vi "Comparaison alarmes 1 2 3 4.vi"() -> (2 "AL OK nouveau":cluster{"AL OK 1 COM":u16[]}[](array[cluster]) {"AL OK 1 COM" items=["data = AL", "data pas nombre", "data diff. AL"]}, 3 "problème":string, 4 "regs pb":string[](array[string]), 5 "Dépassement seuil":T1(array[cluster]))   [LabVIEW 2022 SP3]
uses:
  Variables globales/Variables glob EUROTHERM.vi
panel:
  # "COMPARAISON"
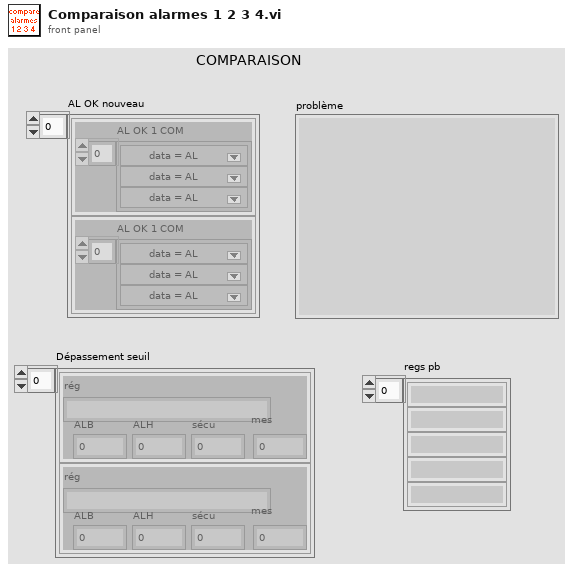
[diagram p1: front panel]
types:
  T1 = cluster{"rég":string, "mes":dbl, "ALB":dbl, "ALH":dbl, "sécu":dbl}[]
  T2 = cluster{"Noms voies select acqui 1COM":string[]}[]
  T3 = cluster{"rég":string, "mes":dbl, "ALB":dbl, "ALH":dbl, "sécu":dbl}
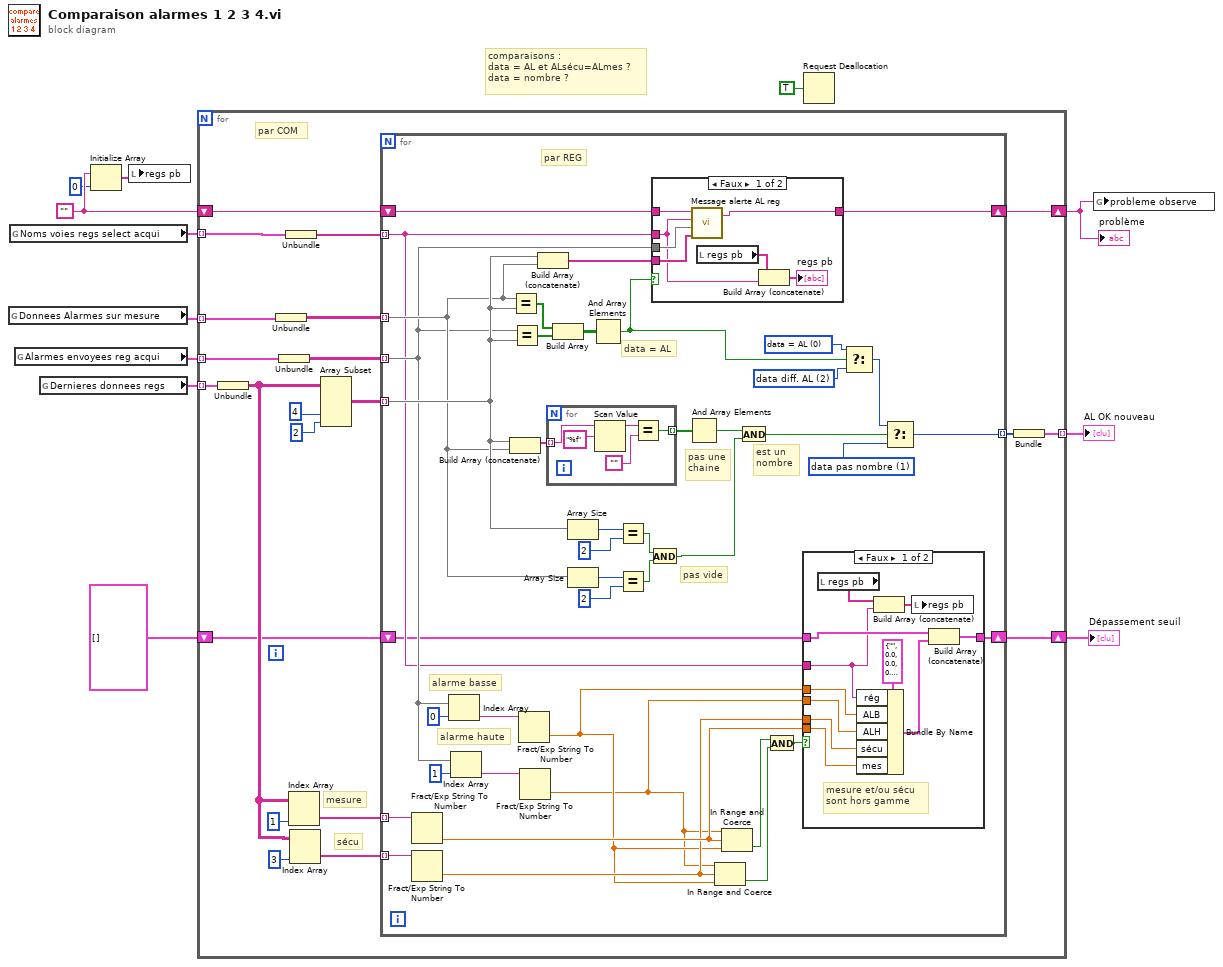
[diagram p0: block diagram]
diagram:
  w3 = ""
  # "comparaisons :\ndata = AL et ALsécu=ALmes ?\ndata = nombre ?"
  n1 = global read "Variables glob EUROTHERM.vi" "Donnees Alarmes sur mesure"() -> (w6:cluster{"AL sur mes 1COM":string[][]}[])
  n2 = global read "Variables glob EUROTHERM.vi" "Noms voies regs select acqui"() -> (w9:T2)
  n3 = global read "Variables glob EUROTHERM.vi" "Alarmes envoyees reg acqui"() -> (w11:cluster{"alarmes 1COM reg":string[][]}[])
  n4 = global read "Variables glob EUROTHERM.vi" "Dernieres donnees regs"() -> (w12:cluster{"Dernieres donnees 1COM":string[][]}[])
  n5 = Initialize Array(w3, 0 ("taille de la dimension")) -> (w2:string[])
  n6 = local write "regs pb"(w2) -> ()
  n7 = for {
    tunnel: w11 -> [w31] mode=indexing
    tunnel: w12 -> [w30] mode=indexing
    tunnel: w9 -> [w27] mode=indexing
    shift-right: [w24] -> w8
    shift-left: w3 -> [w25]
    tunnel: [w22] -> w7 mode=indexing
    tunnel: w6 -> [w21] mode=indexing
    shift-right: [w15] -> w5
    shift-left: T1 [] ("Dépassement seuil") -> [w16]
    # "sécu"
    # "mesure"
    # "par COM"
    n8 = Unbundle(w30) -> ("Dernieres donnees 1COM"=w19:string[][])
    n9 = Unbundle(w21) -> ("AL sur mes 1COM"=w20:string[][])
    n10 = Unbundle(w31) -> ("alarmes 1COM reg"=w29:string[][])
    n11 = Unbundle(w27) -> ("Noms voies select acqui 1COM"=w26:string[])
    n12 = Index Array(array=w19, index (col)=1 ("indice (ligne)")) -> (element=w18:string[])  [unwired: 1 in]
    n13 = Index Array(array=w19, index (col)=3 ("indice (ligne)")) -> (element=w17:string[])  [unwired: 1 in]
    n14 = Array Subset(array=w19, index (col)=4 ("indice"), length (col)=2 ("longueur")) -> (w28:string[][])  [unwired: 2 in]
    n15 = for {
      tunnel: w29 -> [w48] mode=indexing
      tunnel: w28 -> [w53] mode=indexing
      tunnel: w26 -> [w43] mode=indexing
      tunnel: [w63] -> w23 mode=indexing
      shift-right: [w71] -> w24
      shift-left: w25 -> [w70]
      tunnel: w20 -> [w52] mode=indexing
      tunnel: w18 -> [w44] mode=indexing
      tunnel: w17 -> [w45] mode=indexing
      shift-right: [w36] -> w15
      shift-left: w16 -> [w37]
      w65 = u16 2 items=["data = AL", "data pas nombre", "data diff. AL"] ("état AL")
      w66 = u16 0 items=["data = AL", "data pas nombre", "data diff. AL"] ("état AL")
      w68 = u16 1 items=["data = AL", "data pas nombre", "data diff. AL"] ("état AL")
      # "alarme haute"
      # "alarme basse"
      # "par REG"
      # "est un\nnombre"
      # "pas vide"
      # "data = AL"
      # "pas une\nchaine"
      n16 = Fract/Exp String To Number(string=w44) -> (number=w42:dbl)  [unwired: 3 in, 1 out]
      n17 = Fract/Exp String To Number(string=w45) -> (number=w41:dbl)  [unwired: 3 in, 1 out]
      n18 = Index Array(array=w48, index=0 ("indice")) -> (element=w47:string)
      n19 = Index Array(array=w48, index=1 ("indice")) -> (element=w46:string)
      n20 = Build Array (concatenate)(w53, w52) -> (w54:string[])
      n21 = Equal?(x=w52, y=w53) -> (x = y?=w62:bool[])
      n22 = Equal?(x=w48, y=w53) -> (x = y?=w61:bool[])
      n23 = Fract/Exp String To Number(string=w47) -> (number=w35:dbl)  [unwired: 3 in, 1 out]
      n24 = Fract/Exp String To Number(string=w46) -> (number=w34:dbl)  [unwired: 3 in, 1 out]
      n25 = Build Array (concatenate)(w53, w52) -> (w51:string[])
      n26 = for {
        tunnel: w54 -> [w99] mode=indexing
        tunnel: [w96] -> w75 mode=indexing
        n27 = Scan Value(string=w99, format string="%f" ("chaîne de format")) -> (output string=w97:string)  [unwired: 1 in, 1 out]
        n28 = Equal?(x=w97, y="") -> (x = y?=w96:bool)
      }
      n29 = Build Array(w62, w61) -> (w60:bool[][])
      n30 = Array Size(array=w53) -> (size(s)=w74:i32)
      n31 = Array Size(array=w52) -> (size(s)=w58:i32)
      n32 = And Array Elements(Boolean array=w60) -> (logical AND=w67:bool)
      n33 = Equal?(x=w74, y=2) -> (x = y?=w57:bool)
      n34 = Equal?(x=w58, y=2) -> (x = y?=w56:bool)
      n35 = And(x=w57, y=w56) -> (x .and. y?=w55:bool)
      n36 = case shown="Faux" w67 {
        tunnel: w48 -> [w94 _]
        tunnel: w51 -> [w93 _]
        tunnel: w43 -> [w89 _]
        tunnel: [w91 w95] -> w71
        tunnel: w70 -> [w92 w95]
        frame False {
          n37 = call "Message alerte AL reg.vi"("Données alarmes"=w93, "alarmes 1COM reg"=w94, "Noms voies regs sélect acqui 1 COM"=w89, "Message entrée"=w92) -> ("Message sortie"=w91:string)  [unwired: 1 in]
          n38 = local read "regs pb"() -> (w90:string[])
          n39 = Build Array (concatenate)(w90, w89) -> (→"regs pb":string[])
        }
        frame True {
        }
      }
      n40 = And Array Elements(Boolean array=w75) -> (logical AND=w72:bool)
      n41 = In Range and Coerce(upper limit=w34, x=w41, lower limit=w35) -> (In Range?=w39:bool)  [unwired: 1 out]
      n42 = In Range and Coerce(upper limit=w34, x=w42, lower limit=w35) -> (In Range?=w40:bool)  [unwired: 1 out]
      n43 = And(x=w72, y=w55) -> (x .and. y?=w69:bool)
      n44 = And(x=w40, y=w39) -> (x .and. y?=w38:bool)
      n45 = case shown="Faux" w38 {
        tunnel: w43 -> [w77 _]
        tunnel: w34 -> [w82 _]
        tunnel: w35 -> [w83 _]
        tunnel: w42 -> [w80 _]
        tunnel: w41 -> [w81 _]
        tunnel: w37 -> [w85 w87]
        tunnel: [w86 w87] -> w36
        frame False {
          # "mesure et/ou sécu \nsont hors gamme"
          n46 = local read "regs pb"() -> (w78:string[])
          n47 = Bundle By Name(cluster=T3 {"rég"="", "mes"=0.0, "ALB"=0.0, "ALH"=0.0, "sécu"=0.0} ("Cluster"), "rég"=w77, "ALB"=w83, "ALH"=w82, "sécu"=w81, "mes"=w80) -> (w79:T3)
          n48 = Build Array (concatenate)(w78, w77) -> (w76:string[])
          n49 = local write "regs pb"(w76) -> ()
          n50 = Build Array (concatenate)(w85, w79) -> (w86:T1)
        }
        frame True {
          # "mesure et sécu \nne sont pas en alarme"
        }
      }
      n51 = Select(t=w66, s=w67, f=w65) -> (s? t:f=w64:u16)
      n52 = Select(t=w64, s=w69, f=w68) -> (s? t:f=w63:u16)
    }
    n53 = Bundle(w23) -> (w22:cluster{u16[]})  [unwired: 1 in]
  }
  "problème" <- w8
  "AL OK nouveau" <- w7
  "Dépassement seuil" <- w5
  n54 = Request Deallocation(TRUE ("flag")) -> ()
  n55 = global write "Variables glob EUROTHERM.vi" "probleme observe"(w8) -> ()
